vi "getXMLTestCases (Extended).vi"(9 "indent level":i32, 10 "testcases":T1[](array[typedef]), 11 "Test Report in":refnum<class "Test Report.lvclass">) -> (2 "XML Lines":string[](array[string]), 3 "Test Report":refnum<class "Test Report.lvclass">)   [LabVIEW 2020, in "Caraya.lvlib" / "Test Report.JUnit.lvclass"]
uses:
  Test Report.JUnit.lvclass
  extended -- cluster.ctl
  Test Report/Test Report.lvclass
  MsgSerializer.XML/MsgSerializer.XML.lvclass
  C:/projects/caraya/src/classes/MsgSerializer/MsgSerializer.lvclass
  Test Report/Test Report.lvclass/Test Report.ctl
  MsgSerializer/MsgSerializer.lvclass/MsgSerializer.ctl
  MsgSerializer.XML/format -- enum.ctl
  MsgSerializer.XML/MsgSerializer.XML.lvclass/MsgSerializer.XML.ctl
  MsgSerializer/MsgSerializer.lvclass
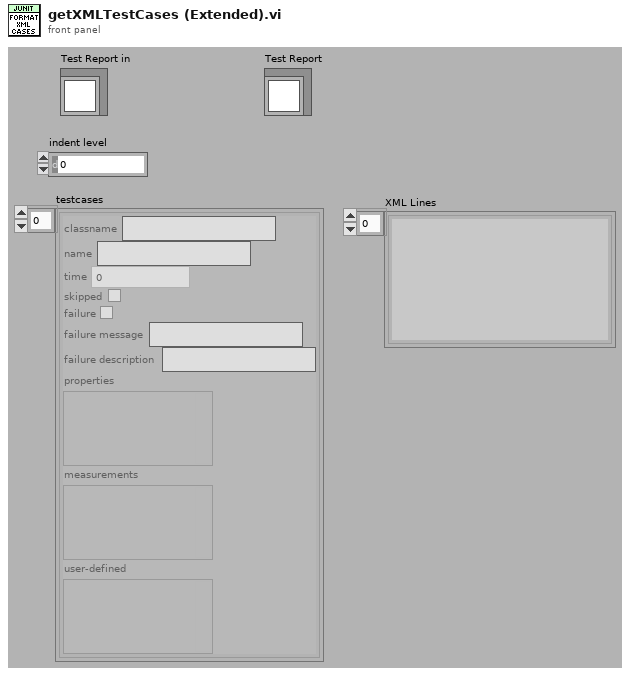
[diagram p1: front panel]
types:
  T1 = typedef "Caraya.lvlib/Test Report.JUnit.lvclass/extended -- cluster.ctl" = cluster{"classname":string, "name":string, "time":dbl, "skipped":bool, "failure":bool, "failure message":string, "failure description":string, "properties":variant, "measurements":variant, "user-defined":variant}
  T2 = typedef "Caraya.lvlib/MsgSerializer.XML.lvclass/format -- enum.ctl" = enum16{"value", "tag", "property"}
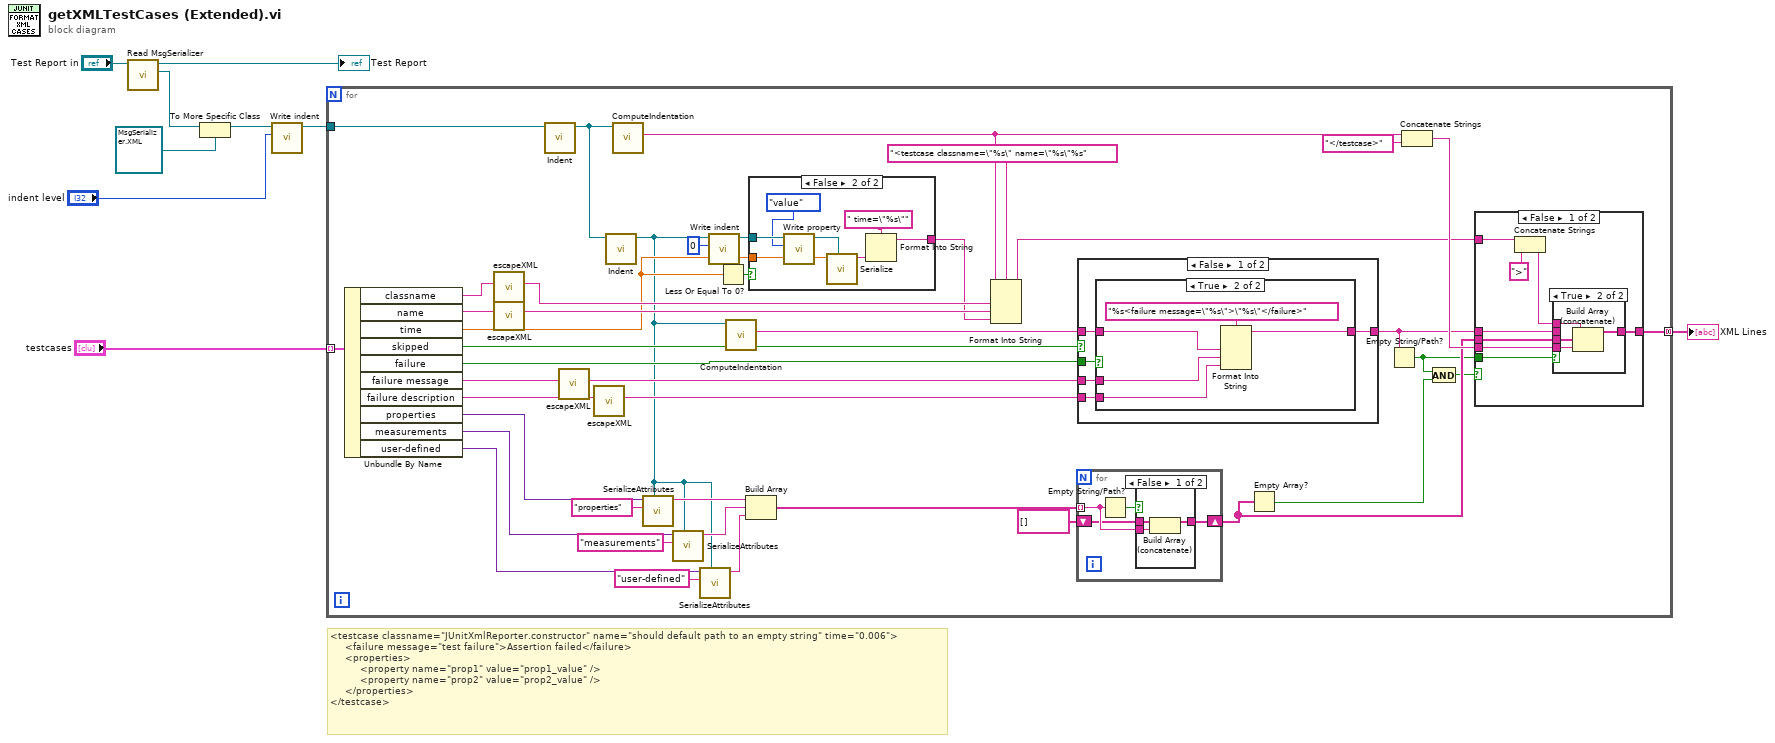
[diagram p0: block diagram]
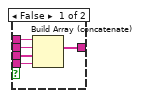
[diagram p4: hidden frame]
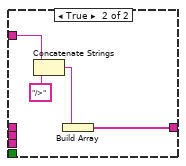
[diagram p5: hidden frame]
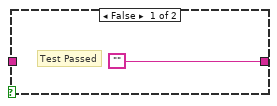
[diagram p6: hidden frame]
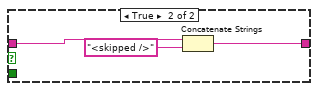
[diagram p7: hidden frame]
diagram:
  # "<testcase classname=\"JUnitXmlReporter.constructor\" name=\"should default path to an empty string\" time=\"0.006\">\n     <failure message=\"test failure\">Assertion failed</failure>\n     <properties>\n          <property name=\"prop1\" value=\"prop1_value\" />\n          <property name=\"prop2\" value=\"prop2_value\" />\n     </properties>\n</testcase>"
  n1 = call "Read MsgSerializer.vi"("Test Report in"="Test Report in") -> ("MsgSerializer"=w3:refnum<class "MsgSerializer.lvclass">, "Test Report out"=→"Test Report":refnum<class "Test Report.lvclass">)  [unwired: 9 in]
  n2 = To More Specific Class(target class=refnum<class "MsgSerializer.XML.lvclass"> refnum ("MsgSerializer"), reference=w3) -> (specific class reference=w2:refnum<class "MsgSerializer.XML.lvclass">)  [unwired: 1 in, 1 out]
  n3 = call "Write indent.vi"("indent"="indent level", "MsgSerializer in"=w2) -> ("MsgSerializer out"=w5:refnum<class "MsgSerializer.XML.lvclass">)  [unwired: 9 in]
  n4 = for {
    tunnel: "testcases" -> [w51] mode=indexing
    tunnel: [w20] -> w8 mode=concatenating
    tunnel: w5 -> [w29]
    n5 = Unbundle By Name(w51) -> ("classname"=w48:string, "name"=w46:string, "time"=w14:dbl, "skipped"=w50:bool, "failure"=w49:bool, "failure message"=w44:string, "failure description"=w42:string, "properties"=w36:variant, "measurements"=w38:variant, "user-defined"=w33:variant)
    n6 = call "escapeXML.vi"("Input String"=w48) -> ("XML-escaped String"=w47:string)  [unwired: 10 in]
    n7 = call "escapeXML.vi"("Input String"=w46) -> ("XML-escaped String"=w45:string)  [unwired: 10 in]
    n8 = call "Indent.vi"("MsgSerializer in"=w29) -> ("MsgSerializer out"=w28:refnum<class "MsgSerializer.XML.lvclass">)  [unwired: 10 in]
    n9 = call "escapeXML.vi"("Input String"=w44) -> ("XML-escaped String"=w43:string)  [unwired: 10 in]
    n10 = call "escapeXML.vi"("Input String"=w42) -> ("XML-escaped String"=w41:string)  [unwired: 10 in]
    n11 = call "Indent.vi"("MsgSerializer in"=w28) -> ("MsgSerializer out"=w10:refnum<class "MsgSerializer.XML.lvclass">)  [unwired: 10 in]
    n12 = call "ComputeIndentation.vi"("MsgSerializer in"=w28) -> ("indentation"=w12:string)  [unwired: 10 in]
    n13 = call "SerializeAttributes.vi"("MsgSerializer"=w10, "attribute name"="properties", "variant attribute"=w36) -> ("Serialized Message"=w26:string)  [unwired: 8 in]
    n14 = call "SerializeAttributes.vi"("MsgSerializer"=w10, "attribute name"="measurements", "variant attribute"=w38) -> ("Serialized Message"=w25:string)  [unwired: 8 in]
    n15 = call "SerializeAttributes.vi"("MsgSerializer"=w10, "attribute name"="user-defined", "variant attribute"=w33) -> ("Serialized Message"=w24:string)  [unwired: 8 in]
    n16 = call "Write indent.vi"("indent"=0, "MsgSerializer in"=w10) -> ("MsgSerializer out"=w13:refnum<class "MsgSerializer.XML.lvclass">)  [unwired: 9 in]
    n17 = Less Or Equal To 0?(x=w14) -> (x <= 0?=w31:bool)
    n18 = call "ComputeIndentation.vi"("MsgSerializer in"=w10) -> ("indentation"=w27:string)  [unwired: 10 in]
    n19 = Build Array(w26, w25, w24) -> (w22:string[])
    n20 = case shown="False" w31 {
      tunnel: [_ w65] -> w32
      tunnel: w14 -> [_ w64]
      tunnel: w13 -> [_ w62]
      frame True {
      }
      frame False {
        n21 = call "Write property.vi"("format"=format_--_enum."value", "MsgSerializer.XMLProperty in"=w62) -> ("MsgSerializer.XMLProperty out"=w61:refnum<class "MsgSerializer.XML.lvclass">)  [unwired: 9 in]
        n22 = call-dynamic "Serialize.vi"("MsgSerializer"=w61, "Value"=w64) -> ("Serialized Message"=w63:string)  [unwired: 8 in, 1 out]
        n23 = Format Into String(format string=" time=\"%s\"", w63) -> (resulting string=w65:string)  [unwired: 2 in, 1 out]
      }
    }
    n24 = Format Into String(format string="<testcase classname=\"%s\" name=\"%s\"%s", initial string=w12, w47, w45, w32) -> (resulting string=w15:string)  [unwired: 1 in, 1 out]
    n25 = for {
      shift-right: [w53] -> w21
      shift-left: string[] [] -> [w54]
      tunnel: w22 -> [w55] mode=indexing
      n26 = Empty String/Path?(string/path=w55) -> (empty?=w52:bool)
      n27 = case shown="False" w52 {
        tunnel: [w58 w59] -> w53
        tunnel: w54 -> [w57 w59]
        tunnel: w55 -> [w56 _]
        frame False {
          n28 = Build Array (concatenate)(w57, w56) -> (w58:string[])
        }
        frame True {
        }
      }
    }
    n29 = case shown="False" w50 {
      tunnel: w49 -> [w92 _]
      tunnel: w43 -> [w91 _]
      tunnel: w41 -> [w90 _]
      tunnel: w27 -> [w89 w100]
      tunnel: [w88 w99] -> w16
      frame False {
        n30 = case shown="True" w92 {
          tunnel: w91 -> [_ w97]
          tunnel: w90 -> [_ w96]
          tunnel: w89 -> [_ w95]
          tunnel: ["" w94] -> w88
          frame False {
            # "Test Passed"
          }
          frame True {
            n31 = Format Into String(format string="%s<failure message=\"%s\">\"%s\"</failure>", w95, w97, w96) -> (resulting string=w94:string)  [unwired: 2 in, 1 out]
          }
        }
      }
      frame True {
        n32 = Concatenate Strings(w100, "<skipped />") -> (w99:string)
      }
    }
    n33 = Empty Array?(array=w21) -> (empty?=w19:bool)
    n34 = Empty String/Path?(string/path=w16) -> (empty?=w17:bool)
    n35 = Concatenate Strings(w12, "</testcase>") -> (w39:string)
    n36 = And(x=w17, y=w19) -> (x .and. y?=w18:bool)
    n37 = case shown="False" w18 {
      tunnel: w15 -> [w73 w85]
      tunnel: [w70 w84] -> w20
      tunnel: w39 -> [w69 _]
      tunnel: w16 -> [w71 _]
      tunnel: w21 -> [w68 _]
      tunnel: w17 -> [w67 _]
      frame False {
        n38 = Concatenate Strings(w73, ">" ("string")) -> (w72:string)
        n39 = case shown="True" w67 {
          tunnel: w72 -> [w79 w81]
          tunnel: w71 -> [w78 _]
          tunnel: [w77 w80] -> w70
          tunnel: w69 -> [w76 w83]
          tunnel: w68 -> [w75 w82]
          frame False {
            n40 = Build Array (concatenate)(w79, w78, w75, w76) -> (w77:string[])
          }
          frame True {
            n41 = Build Array (concatenate)(w81, w82, w83) -> (w80:string[])
          }
        }
      }
      frame True {
        n42 = Concatenate Strings(w85, "/>" ("string")) -> (w87:string)
        n43 = Build Array(w87) -> (w84:string[])
      }
    }
  }
  "XML Lines" <- w8
